vi "VIH HelpGen - Get Target HTML Filename - Make Name.vi"(10 "Item Filename":string) -> (2 "HTML Filename":string)   [LabVIEW 2014]
doc: "::: VI Helpeks :::\nCopyright (c) 2000-2026 Konstantin Shifershteyn. All rights reserved."
panel:
  # "VI Helpeks\nCopyright (c) 2012-2026 Konstantin Shifershteyn"
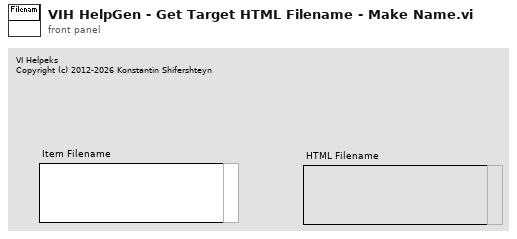
[diagram p1: front panel]
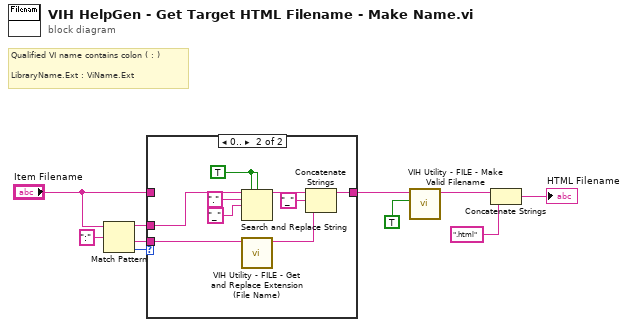
[diagram p0: block diagram]
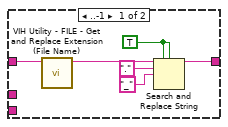
[diagram p2: hidden frame]
diagram:
  # "Qualified VI name contains colon ( : )\n\nLibraryName.Ext : ViName.Ext"
  n1 = Match Pattern(string="Item Filename", regular expression=":") -> (before substring=w6:string, after substring=w7:string, offset past match=w9:i32)  [unwired: 1 in, 1 out]
  n2 = case shown="0.." w9 {
    tunnel: "Item Filename" -> [w16 _]
    tunnel: [w11 w24] -> w5
    tunnel: w7 -> [_ w18]
    tunnel: w6 -> [_ w19]
    frame ..-1 {
      w13 = TRUE
      n3 = call "VIH Utility - FILE - Get and Replace Extension (File Name).vi"("File name"=w16) -> ("File name out"=w12:string)  [unwired: 9 in, 1 out]
      n4 = Search and Replace String(replace all?=w13, case sensitive?=w13, input string=w12, search string=".", replace string="_" ("replace string (\"\")")) -> (result string=w11:string)  [unwired: 3 in, 3 out]
    }
    frame 0.. {
      w21 = TRUE
      n5 = Search and Replace String(replace all?=w21, case sensitive?=w21, input string=w19, search string=".", replace string="_" ("replace string (\"\")")) -> (result string=w20:string)  [unwired: 3 in, 3 out]
      n6 = call "VIH Utility - FILE - Get and Replace Extension (File Name).vi"("File name"=w18) -> ("File name out"=w17:string)  [unwired: 9 in, 1 out]
      n7 = Concatenate Strings(w20, "_" ("string"), w17) -> (w24:string)
    }
  }
  n8 = call "VIH Utility - FILE - Make Valid Filename.vi"("comply to CHM (F)"=TRUE, "File Name in"=w5) -> ("File Name out"=w1:string)  [unwired: 9 in]
  n9 = Concatenate Strings(w1, ".html") -> (→"HTML Filename":string)
